vi "Tester.vi"() -> ()   [LabVIEW 2025, in "G-Uart-Class.lvclass"]
uses:
  G-Uart-Class.lvclass
panel:
  in  "路径":path
  in  "停止":bool
  # "c测试串口使用"
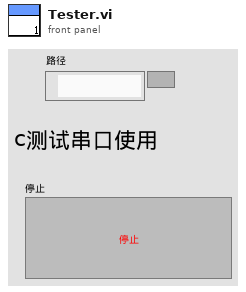
[diagram p1: front panel]
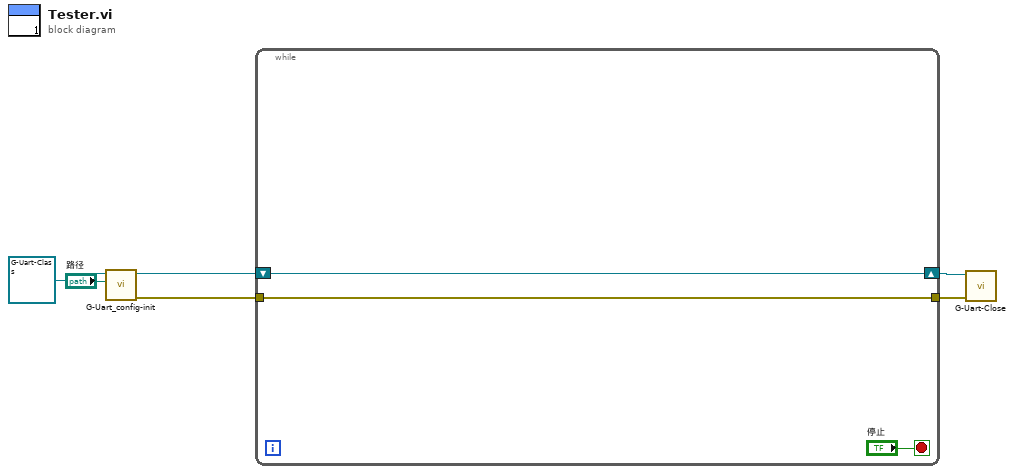
[diagram p0: block diagram]
diagram:
  n1 = call-dynamic "G-Uart_config-init.vi"("路径"="路径", "G-Uart-Class 输入"=refnum<class "G-Uart-Class.lvclass"> refnum ("G-Uart-Class.lvclass")) -> ("error out"=w4:errorcluster, "G-Uart-Class 输出"=w2:refnum<class "G-Uart-Class.lvclass">)  [unwired: 8 in]
  n2 = while {
    shift-right: [w8] -> w5
    shift-left: w2 -> [w8]
    tunnel: w4 -> [w7]
    tunnel: [w7] -> w3
    stop <- "停止" stop-if-true
  }
  n3 = call-dynamic "G-Uart-Close.vi"("error in (no error)"=w3, "G-Uart-Class 输入"=w5) -> ()  [unwired: 8 in, 2 out]
